vi "Test_Send_Apply_Setpoints.vi"(10 "setpoints":cluster{"channel":string, "value":dbl}[](array[cluster]), 11 "class path":path) -> (0 "error out":errorcluster)   [LabVIEW 2026]
doc: "Manual smoke test for Apply Setpoints Msg: load the VTU Sim Rig class from a path, cast to Actor, launch it as a root actor, send Apply Setpoints with the given setpoints, send Normal Stop, and report the final error out. No error means the Send to Do round trip dispatched and executed cleanly."
uses:
  <vilib>/ActorFramework/Actor/Actor.lvclass
  src/Rig Messages/Apply Setpoints Msg/Apply Setpoints Msg.lvclass/Apply Setpoints Msg.ctl
  <vilib>/ActorFramework/Message Enqueuer/Message Enqueuer.lvclass/Message Enqueuer.ctl
  <vilib>/ActorFramework/Message Enqueuer/Enqueue.vi
  src/Rig Messages/Apply Setpoints Msg/Apply Setpoints Msg.lvclass
  <vilib>/ActorFramework/Stop Msg/Stop Msg.lvclass
  <vilib>/ActorFramework/Message Priority Queue/Priority Enqueue.vi
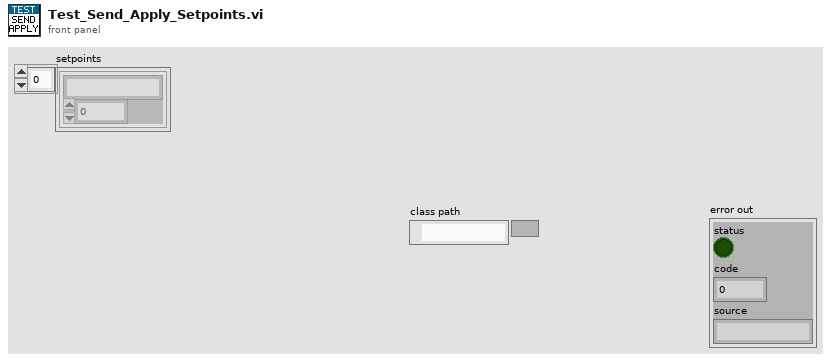
[diagram p1: front panel]
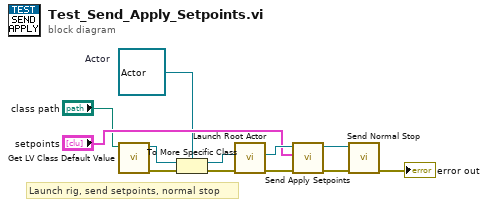
[diagram p0: block diagram]
diagram:
  w1 = refnum<class "Actor.lvclass"> refnum  # Actor
  # "Launch rig, send setpoints, normal stop"
  n1 = call <vilib>:"Get LV Class Default Value.vi"("class path"="class path") -> ("error out"=w5:errorcluster, "object"=w4:refnum<class>)  [unwired: 9 in]
  n2 = To More Specific Class(target class=w1, reference=w4, error in=w5) -> (specific class reference=w6:refnum<class "Actor.lvclass">, error out=w7:errorcluster)
  n3 = call <vilib>:"Launch Root Actor.vi"("error in (no error)"=w7, "Actor"=w6) -> ("error out"=w9:errorcluster, "Actor's Enqueuer"=w8:refnum<class "Message Enqueuer.lvclass">)  [unwired: 8 in]
  n4 = call "Send Apply Setpoints.vi"("error in (no error)"=w9, "setpoints"="setpoints", "Message Enqueuer"=w8) -> ("error out"=w11:errorcluster, "Message Enqueuer out"=w10:refnum<class "Message Enqueuer.lvclass">)  [unwired: 7 in]
  n5 = call <vilib>:"Send Normal Stop.vi"("error in (no error)"=w11, "Message Enqueuer"=w10) -> ("error out"=→"error out":errorcluster)  [unwired: 9 in]
